vi "KeyDown.vi"(6 "PlatMods":T9, 7 "Type":T1, 8 "error in":errorcluster, 9 "VKey":T10, 10 "Char":i16, 11 "Data in":T2={"Class"={"Ants"=refnum, "Layer"=refnum, "Templates"=refnum, "Icon"=refnum, "Glyph"=refnum, "Settings"=refnum, "Tools"=refnum, "History"=refnum}, "Ref"={"Add Layer"=refnum, "Remove Layer"=refnum, "Line Text"=[], "Body Text Spec"=refnum, "DNL_Font"=refnum, "glyph path str"=refnum, "templates path str"=refnum, "Arrow Up"=refnum, "Arrow Down"=refnum, "IE VI Ref"=refnum, "Glyphs tree"=refnum, "Templates tree"=refnum, "Layer Icon Text"=refnum, "Layer Template"=refnum, "Body Text"=refnum, "Search Templates"=refnum, "TextMarker"=refnum, "Tab Control"=refnum, "Search Glyphs"=refnum, "Line Color"=refnum, "DNL_Glyphs []"=refnum, "Fill Color"=refnum, "Tools"=refnum, "Icon"=refnum, "Preview"=refnum, "Ants"=refnum, "Terminals"=refnum, "menu reference"=refnum, "LayerNames"=[], "GlyphLoadAnimation"=refnum, "TemplateLoadAnimation"=refnum, "refreshGlyphs"=refnum, "refreshTemplates"=refnum}, "Support"={"AntsRect"={"left"=0, "top"=0, "right"=0, "bottom"=0}, "Mouse Move Coords"={"Horizontal"=0, "Vertical"=0}, "Mouse Down Coords"={"Horizontal"=0, "Vertical"=0}, "Temp Coord"={"Horizontal"=0, "Vertical"=0}, "Action"=enum."Default", "Edge Color"=4914962, "Fill Color"=16860, "Mouse Down?"=FALSE, "Draft Mode?"=FALSE, "Temp Icon"=bytes[3102], "CTRL Pressed"=FALSE, "Move Selection?"=FALSE, "AntsRect Orig"={"left"=0, "top"=0, "right"=0, "bottom"=0}, "Text"="", "TM Set?"=FALSE, "Mouse inside icon?"=FALSE, "Tool (old value)"=0, "Pencil Move Color"=0, "Swap Colors?"=FALSE, "Shift pressed?"=FALSE}}) -> (0 "error out":errorcluster, 1 "Discard?":bool, 3 "Data out":T2={"Class"={"Ants"=refnum, "Layer"=refnum, "Templates"=refnum, "Icon"=refnum, "Glyph"=refnum, "Settings"=refnum, "Tools"=refnum, "History"=refnum}, "Ref"={"Add Layer"=refnum, "Remove Layer"=refnum, "Line Text"=[], "Body Text Spec"=refnum, "DNL_Font"=refnum, "glyph path str"=refnum, "templates path str"=refnum, "Arrow Up"=refnum, "Arrow Down"=refnum, "IE VI Ref"=refnum, "Glyphs tree"=refnum, "Templates tree"=refnum, "Layer Icon Text"=refnum, "Layer Template"=refnum, "Body Text"=refnum, "Search Templates"=refnum, "TextMarker"=refnum, "Tab Control"=refnum, "Search Glyphs"=refnum, "Line Color"=refnum, "DNL_Glyphs []"=refnum, "Fill Color"=refnum, "Tools"=refnum, "Icon"=refnum, "Preview"=refnum, "Ants"=refnum, "Terminals"=refnum, "menu reference"=refnum, "LayerNames"=[], "GlyphLoadAnimation"=refnum, "TemplateLoadAnimation"=refnum, "refreshGlyphs"=refnum, "refreshTemplates"=refnum}, "Support"={"AntsRect"={"left"=0, "top"=0, "right"=0, "bottom"=0}, "Mouse Move Coords"={"Horizontal"=0, "Vertical"=0}, "Mouse Down Coords"={"Horizontal"=0, "Vertical"=0}, "Temp Coord"={"Horizontal"=0, "Vertical"=0}, "Action"=enum."Default", "Edge Color"=4914962, "Fill Color"=16860, "Mouse Down?"=FALSE, "Draft Mode?"=FALSE, "Temp Icon"=bytes[3102], "CTRL Pressed"=FALSE, "Move Selection?"=FALSE, "AntsRect Orig"={"left"=0, "top"=0, "right"=0, "bottom"=0}, "Text"="", "TM Set?"=FALSE, "Mouse inside icon?"=FALSE, "Tool (old value)"=0, "Pencil Move Color"=0, "Swap Colors?"=FALSE, "Shift pressed?"=FALSE}})   [LabVIEW 2020]
uses:
  Class/Ants/Ants.lvclass
  Class/FakedArray/FakedArray.lvclass
  vi.lib/LabVIEW Icon API/lv_icon/Classes/Icon/Icon.lvclass
  Class/Icon Library/Glyph.lvclass
  Class/Settings/Settings.lvclass
  Class/Tools/Tools Paint.lvclass
  History/History/History.lvclass
  lv_icon.lvlib
  <vilib>/Utility/miscctls.llb/LVPoint32TypeDef.ctl
  <vilib>/event_ctls.llb/lveventtype.ctl
  Controls/SupportClass_Action.ctl
  History/History.lvlib
  <vilib>/event_ctls.llb/eventvkey.ctl
  Controls/Support Cluster.ctl
  Controls/References Cluster.ctl
  Controls/IE Classes.ctl
  Controls/Global Data.ctl
  vi.lib/LabVIEW Icon API/lv_icon/Controls/IEColor.ctl
panel:
  in  "Layer name":string="Clipboard"
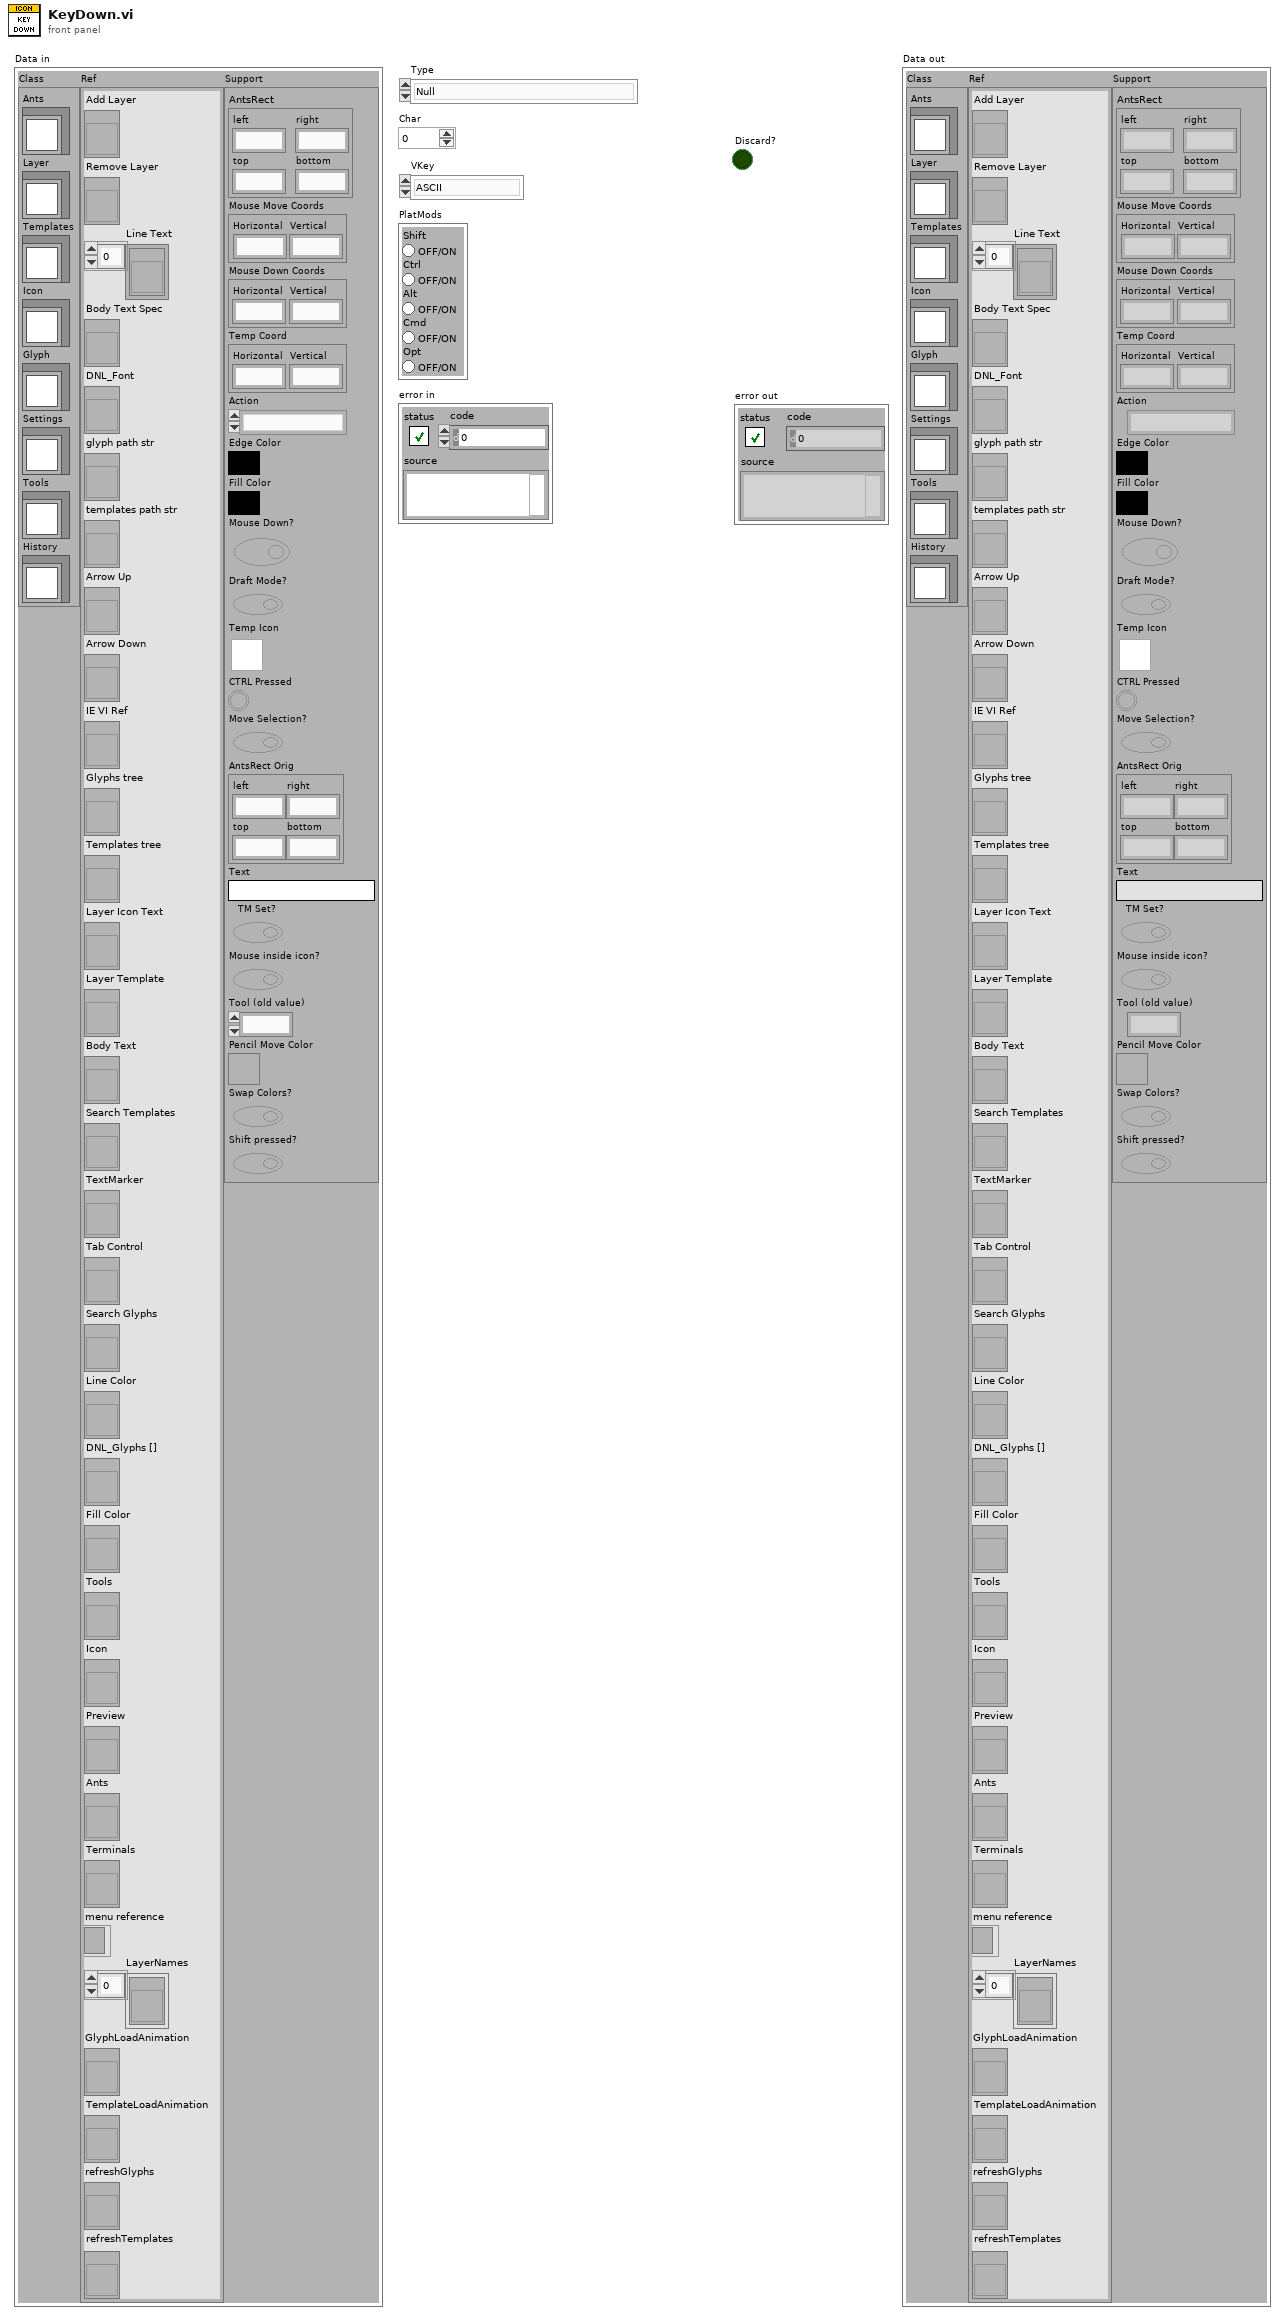
[diagram p1: front panel]
types:
  T1 = typedef "lveventtype.ctl" = enum32{"Null", "Timeout", "Annotation Menu Selection", "Annotation Menu Selection?", "App Instance Close", "App Instance Close?", "Autoscale Range Change", "Bookmark Info Change", "Cell Edit", "Cell Edit?", "Cursor Grab", "Cursor Grab?", "Cursor Menu Selection", "Cursor Menu Selection?", "Cursor Move", "Cursor Release", "Data Change", "Direction Change", "Display State Change", "Drag Ended", "Drag Enter", "Drag Leave", "Drag Over", "Drag Source Update", "Drag Starting", "Drag Starting?", "Drop", "Exec State Change", "Key Down", "Key Down?", "Key Repeat", "Key Repeat?", "Key Up", "Listbox Double Click", "Menu Activation?", "Menu Selection (App)", "Menu Selection? (App)", "Menu Selection (User)", "Mouse Down", "Mouse Down?", "Mouse Enter", "Mouse Leave", "Mouse Move", "Mouse Up", "Mouse Wheel", "NI Security User Change (App)", "Pane Size", "Panel Close", "Panel Close?", "Panel Resize", "Plot Attribute Change", "Scale Range Change", "Shortcut Menu Activation?", "Shortcut Menu Selection (App)", "Shortcut Menu Selection? (App)", "Shortcut Menu Selection (User)", "Tree Double Click", "Tree Drag", "Tree Drag?", "Tree Drop", "Tree Drop?", "Tree Item Close", "Tree Item Close?", "Tree Item Open", "Tree Item Open?", "URL Change?", "User Event", "Value Change"}
  T2 = typedef "lv_icon.lvlib/Global Data.ctl" = cluster{"Class":T3, "Ref":T4, "Support":T5}
  T3 = typedef "lv_icon.lvlib/IE Classes.ctl" = cluster{"Ants":refnum<class "Ants.lvclass">, "Layer":refnum<class "FakedArray.lvclass">, "Templates":refnum<class "FakedArray.lvclass">, "Icon":refnum<class "Icon.lvclass">, "Glyph":refnum<class "Glyph.lvclass">, "Settings":refnum<class "Settings.lvclass">, "Tools":refnum<class "Tools Paint.lvclass">, "History":refnum<class "History.lvclass">}
  T4 = typedef "lv_icon.lvlib/References Cluster.ctl" = cluster{"Add Layer":refnum<vi>, "Remove Layer":refnum<vi>, "Line Text":refnum<vi>[], "Body Text Spec":refnum<vi>, "DNL_Font":refnum<vi>, "glyph path str":refnum<vi>, "templates path str":refnum<vi>, "Arrow Up":refnum<vi>, "Arrow Down":refnum<vi>, "IE VI Ref":refnum<vi>, "Glyphs tree":refnum<vi>, "Templates tree":refnum<vi>, "Layer Icon Text":refnum<vi>, "Layer Template":refnum<vi>, "Body Text":refnum<vi>, "Search Templates":refnum<vi>, "TextMarker":refnum<vi>, "Tab Control":refnum<vi>, "Search Glyphs":refnum<vi>, "Line Color":refnum<vi>, "DNL_Glyphs []":refnum<vi>, "Fill Color":refnum<vi>, "Tools":refnum<vi>, "Icon":refnum<vi>, "Preview":refnum<vi>, "Ants":refnum<vi>, "Terminals":refnum<vi>, "menu reference":refnum<k9>, "LayerNames":refnum<vi>[], "GlyphLoadAnimation":refnum<vi>, "TemplateLoadAnimation":refnum<vi>, "refreshGlyphs":refnum<vi>, "refreshTemplates":refnum<vi>}
  T5 = typedef "lv_icon.lvlib/Support Cluster.ctl" = cluster{"AntsRect":cluster{"left":i16, "top":i16, "right":i16, "bottom":i16}, "Mouse Move Coords":T6, "Mouse Down Coords":T6, "Temp Coord":T6, "Action":T7, "Edge Color":T8, "Fill Color":T8, "Mouse Down?":bool, "Draft Mode?":bool, "Temp Icon":picture, "CTRL Pressed":bool, "Move Selection?":bool, "AntsRect Orig":cluster{"left":i16, "top":i16, "right":i16, "bottom":i16}, "Text":string, "TM Set?":bool, "Mouse inside icon?":bool, "Tool (old value)":u32, "Pencil Move Color":u32, "Swap Colors?":bool, "Shift pressed?":bool}
  T6 = typedef "LVPoint32TypeDef.ctl" = cluster{"Horizontal":i32, "Vertical":i32}
  T7 = typedef "SupportClass_Action.ctl" = enum16{"Default", "Move Selection", "Glyph Library", "Tool"}
  T8 = typedef "IEColor.ctl" = u32
  T9 = cluster{"Shift":bool, "Ctrl":bool, "Alt":bool, "Cmd":bool, "Opt":bool}
  T10 = typedef "eventvkey.ctl" = enum16{"ASCII", "Enter", "Return", "Shift", "Ctrl", "Alt", "Cmd", "Opt", "Caps", "NumLock", "Clear", "Break", "Up", "Down", "Left", "Right", "Insert", "Delete", "Home", "End", "PageUp", "PageDown", "Escape", "Help", "Pause", "ScrollLock", "F1", "F2", "F3", "F4", "F5", "F6", "F7", "F8", "F9", "F10", "F11", "F12", "F13", "F14", "F15", "F16", "F17", "F18", "F19", "F20", "F21", "F22", "F23", "F24", "Play", "VolumeUp", "VolumeDown", "Mute", "Two Byte Char"}
  T11 = cluster{"left":i16, "top":i16, "right":i16, "bottom":i16}
  T12 = enum32{"Pencil", "Line", "Dropper", "Fill", "Rectangle", "Filled Rectangle", "Ellipse", "Filled Ellipse", "Eraser", "Text", "Select", "Move"}
  T13 = typedef "Graphic.ctl" = cluster{"Rectangle":cluster{"left":i16, "top":i16, "right":i16, "bottom":i16}, "Path":path, "Image":picture, "Filter":string, "FileName":string}
  T14 = cluster{"left":i16, "top":i16, "bottom":i16, "right":i16}
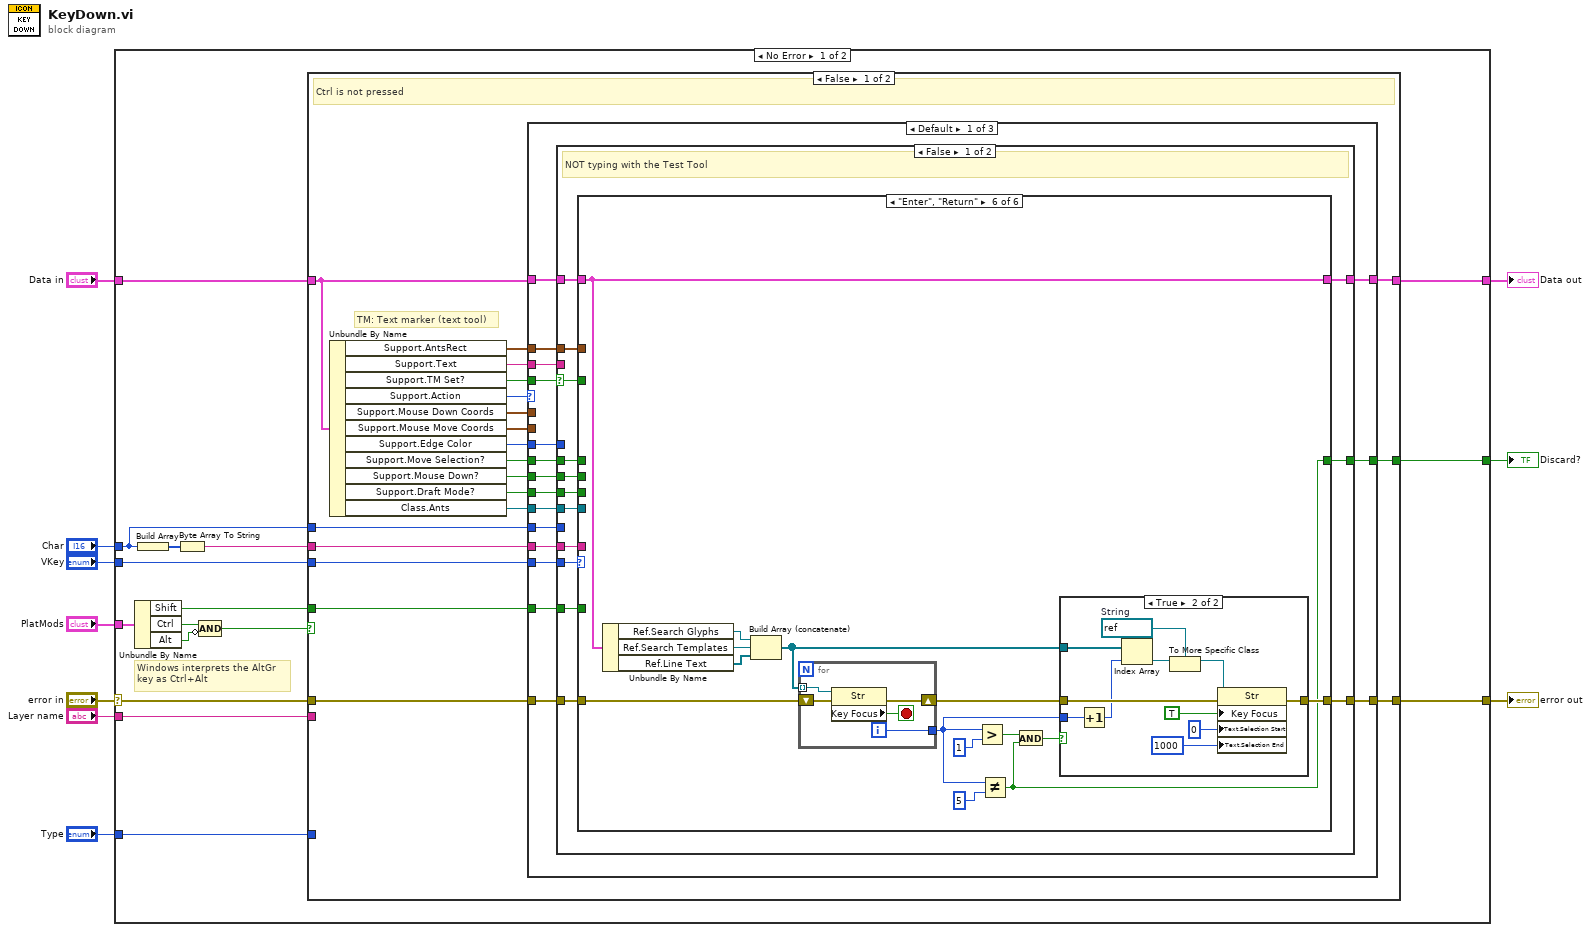
[diagram p0: block diagram]
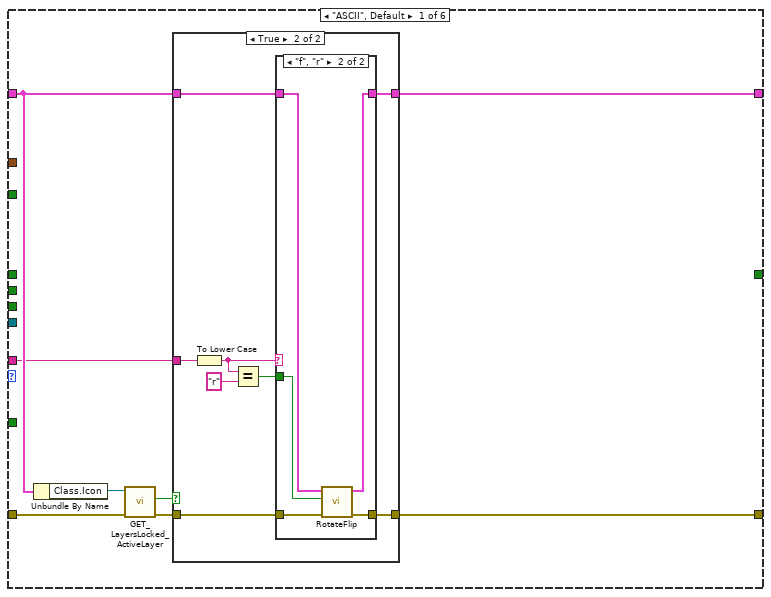
[diagram p2: hidden frame]
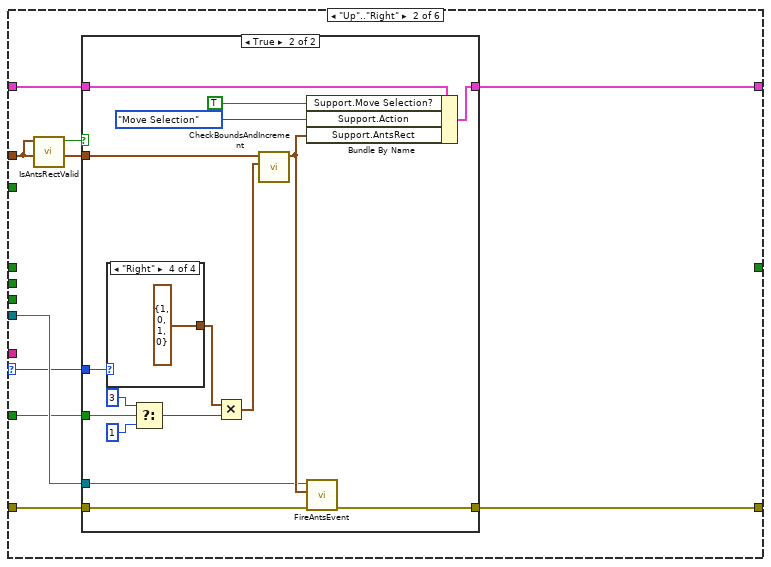
[diagram p5: hidden frame]
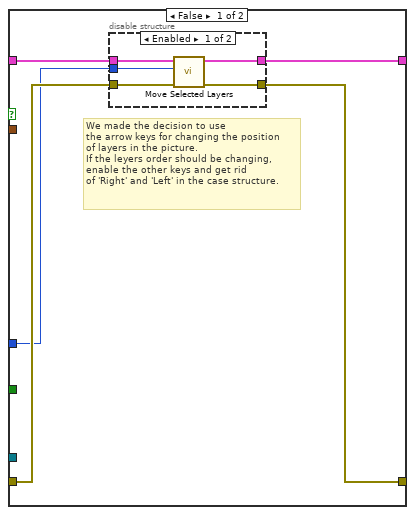
[diagram p6: hidden frame]
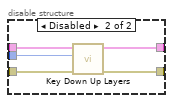
[diagram p7: hidden frame]
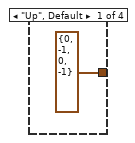
[diagram p8: hidden frame]
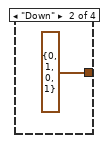
[diagram p9: hidden frame]
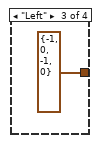
[diagram p10: hidden frame]
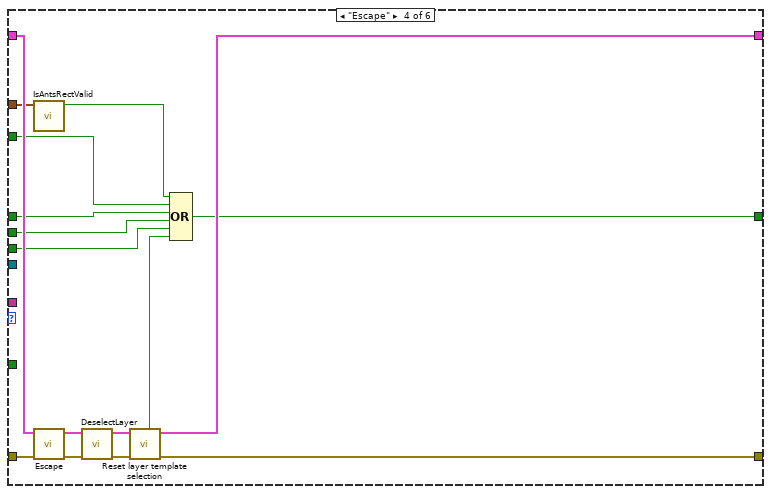
[diagram p12: hidden frame]
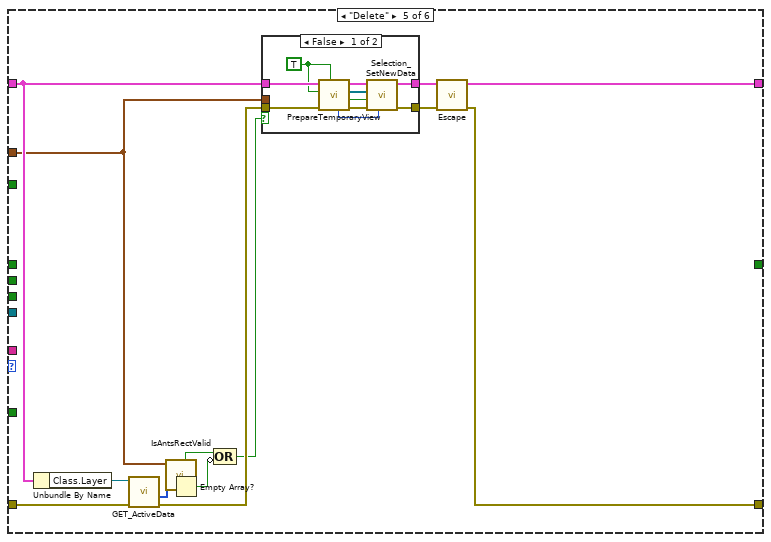
[diagram p13: hidden frame]
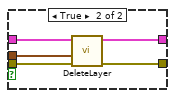
[diagram p14: hidden frame]
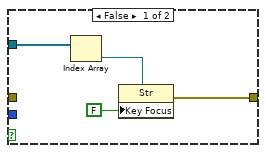
[diagram p15: hidden frame]
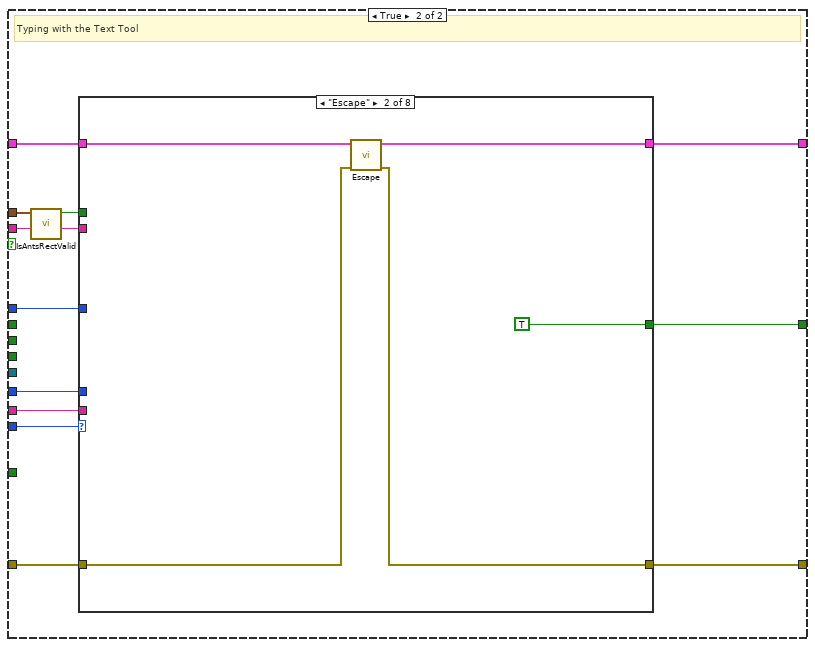
[diagram p16: hidden frame]
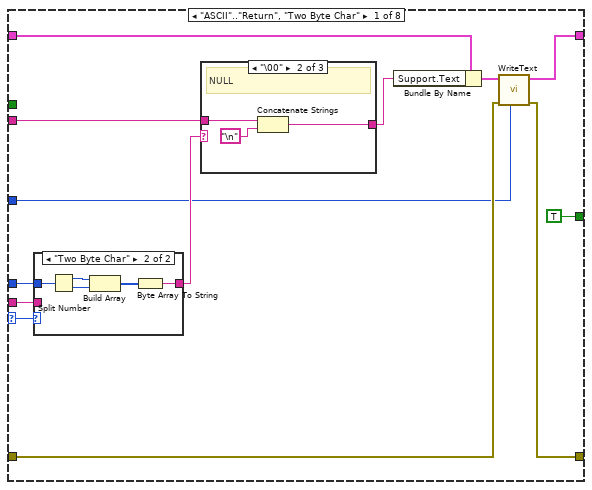
[diagram p17: hidden frame]
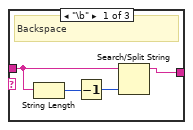
[diagram p19: hidden frame]
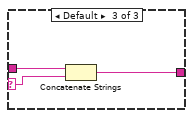
[diagram p20: hidden frame]
diagram:
  n1 = case shown="No Error" "error in" {
    selector: "error in" -> [w25 w688]
    tunnel: [w26 w688] -> w9
    tunnel: "VKey" -> [w24 _]
    tunnel: "Char" -> [w18 _]
    tunnel: "PlatMods" -> [w15 _]
    tunnel: [w21 _] -> w5
    tunnel: "Data in" -> [w16 w687]
    tunnel: [w20 w687] -> w3
    tunnel: "Type" -> [w19 _]
    tunnel: "Layer name" -> [w17 _]
    frame No Error {
      # "Windows interprets the AltGr\nkey as Ctrl+Alt"
      n2 = Unbundle By Name(w15) -> ("Shift"=w11:bool, "Ctrl"=w12:bool, "Alt"=w14:bool)
      n3 = Build Array(w18) -> (w23:i16[])
      n4 = Byte Array To String(unsigned byte array=w23) -> (string=w22:string)
      n5 = Compound Arithmetic op=AND(w12, invert w14) -> (w13:bool)
      n6 = case shown="False" w13 {
        selector: w13 -> [_ w489]
        tunnel: w24 -> [w44 _]
        tunnel: w22 -> [w43 w487]
        tunnel: [w45 w499] -> w26
        tunnel: [w32 w486] -> w21
        tunnel: w25 -> [w46 w500]
        tunnel: w16 -> [w31 w481]
        tunnel: [w29 w498] -> w20
        tunnel: w19 -> [_ w493]
        tunnel: w18 -> [w28 _]
        tunnel: w17 -> [_ w484]
        tunnel: w11 -> [w27 w482]
        frame False {
          # "TM: Text marker (text tool)"
          # "Ctrl is not pressed"
          n7 = Unbundle By Name(w31) -> ("Support.AntsRect"=w37:T11, "Support.Text"=w40:string, "Support.TM Set?"=w41:bool, "Support.Action"=w42:T7, "Support.Mouse Down Coords"=w39:T6, "Support.Mouse Move Coords"=w36:T6, "Support.Edge Color"=w38:T8, "Support.Move Selection?"=w35:bool, "Support.Mouse Down?"=w34:bool, "Support.Draft Mode?"=w33:bool, "Class.Ants"=w30:refnum<class "Ants.lvclass">)
          n8 = case shown="Default" w42 {
            tunnel: w44 -> [w61 w333 w400]
            tunnel: w43 -> [w58 w332 _]
            tunnel: w46 -> [w62 w335 w402]
            tunnel: [w63 w334 w401] -> w45
            tunnel: w41 -> [w60 w330 w398]
            tunnel: w40 -> [w59 _ _]
            tunnel: w39 -> [_ _ _]
            tunnel: w38 -> [w57 _ _]
            tunnel: w37 -> [w56 w331 w399]
            tunnel: w36 -> [_ w323 _]
            tunnel: w35 -> [w55 w329 w397]
            tunnel: w34 -> [w54 w328 w396]
            tunnel: w33 -> [w53 w327 w395]
            tunnel: [w52 w326 w394] -> w32
            tunnel: w27 -> [w51 _ w390]
            tunnel: w31 -> [w50 w325 w393]
            tunnel: [w49 w324 w392] -> w29
            tunnel: w30 -> [w47 _ w391]
            tunnel: w28 -> [w48 _ _]
            frame Default {
              n9 = case shown="False" w60 {
                selector: w60 -> [w69 _]
                tunnel: w61 -> [w75 w236]
                tunnel: [w76 w238] -> w63
                tunnel: w62 -> [w77 w237]
                tunnel: w59 -> [_ w235]
                tunnel: w58 -> [w74 w234]
                tunnel: w57 -> [_ w231]
                tunnel: w56 -> [w73 w233]
                tunnel: w55 -> [w72 _]
                tunnel: w54 -> [w71 _]
                tunnel: w53 -> [w70 _]
                tunnel: [w68 w230] -> w52
                tunnel: w51 -> [w67 _]
                tunnel: w50 -> [w66 w229]
                tunnel: [w65 w228] -> w49
                tunnel: w48 -> [_ w227]
                tunnel: w47 -> [w64 _]
                frame False {
                  # "NOT typing with the Test Tool"
                  n10 = case shown="\"Enter\", \"Return\"" w75 {
                    selector: w75 -> [_ w108 _ _ _ _]
                    tunnel: w77 -> [w84 w111 w148 w164 w175 w206]
                    tunnel: [w85 w110 w148 w161 w177 w204] -> w76
                    tunnel: w74 -> [w78 _ _ _ _ _]
                    tunnel: w73 -> [_ w103 _ w158 w165 _]
                    tunnel: w72 -> [_ _ _ w156 _ _]
                    tunnel: w71 -> [_ _ _ w155 _ _]
                    tunnel: w70 -> [_ _ _ w154 _ _]
                    tunnel: w69 -> [_ _ _ w157 _ _]
                    tunnel: [_ _ _ w149 _ w194] -> w68
                    tunnel: w67 -> [_ w107 _ _ _ _]
                    tunnel: w66 -> [w82 w106 w147 w160 w171 w203]
                    tunnel: [w81 w105 w147 w151 w173 w203] -> w65
                    tunnel: w64 -> [_ w109 _ _ _ _]
                    frame "ASCII", Default {
                      n11 = Unbundle By Name(w82) -> ("Class.Icon"=w80:refnum<class "Icon.lvclass">)
                      n12 = call-dynamic "GET_LayersLocked_ActiveLayer.vi"("error in (no error)"=w84, "Icon.lvclass in"=w80) -> ("error out"=w83:errorcluster, "Layers Locked?"=w79:bool)  [unwired: 8 out]
                      n13 = case shown="True" w79 {
                        tunnel: w78 -> [_ w92]
                        tunnel: w83 -> [w87 w95]
                        tunnel: [w87 w94] -> w85
                        tunnel: w82 -> [w86 w89]
                        tunnel: [w86 w88] -> w81
                        frame False {
                        }
                        frame True {
                          n14 = To Lower Case(string=w92) -> (all lower case string=w90:string)
                          n15 = Equal?(x=w90, y="r") -> (x = y?=w91:bool)
                          n16 = case shown="\"f\", \"r\"" w90 {
                            tunnel: w95 -> [w97 w102]
                            tunnel: [w97 w101] -> w94
                            tunnel: w91 -> [_ w100]
                            tunnel: w89 -> [w96 w99]
                            tunnel: [w96 w98] -> w88
                            frame Default {
                            }
                            frame "f", "r" {
                              n17 = call "RotateFlip.vi"("error in"=w102, "Rotate"=w100, "Data in"=w99) -> ("error out"=w101:errorcluster, "Data out"=w98:T2)  [unwired: 3 in, 4 out]
                            }
                          }
                        }
                      }
                    }
                    frame "Up".."Right" {
                      n18 = call "IsAntsRectValid.vi"("AntsRect"=w103) -> ("Valid?"=w104:bool)  [unwired: 10 out]
                      n19 = case shown="True" w104 {
                        tunnel: w111 -> [w116 w141]
                        tunnel: [w115 w142] -> w110
                        tunnel: w108 -> [w114 w130]
                        tunnel: w107 -> [_ w129]
                        tunnel: w106 -> [w113 w138]
                        tunnel: [w112 w136] -> w105
                        tunnel: w103 -> [_ w127]
                        tunnel: w109 -> [_ w128]
                        frame False {
                          # "We made the decision to use\nthe arrow keys for changing the position\nof layers in the picture.\nIf the leyers order should be changing,\nenable the other keys and get rid\nof 'Right' and 'Left' in the case structure."
                          n20 = disable-structure shown="Enabled" {
                            disable-tunnel: w116 -> [w121 w126]
                            disable-tunnel: [w120 w125] -> w115
                            disable-tunnel: w114 -> [w117 w122]
                            disable-tunnel: w113 -> [w119 w124]
                            disable-tunnel: [w118 w123] -> w112
                            frame Enabled {
                              n21 = call "Move Selected Layers.vi"("error in"=w121, "VKey"=w117, "Data in"=w119) -> ("error out"=w120:errorcluster, "Data out"=w118:T2)  [unwired: 1 in, 6 out]
                            }
                            frame Disabled {
                              n22 = call "Key Down Up Layers.vi"("error in"=w126, "VKey"=w122, "Data in"=w124) -> ("error out"=w125:errorcluster, "Data out"=w123:T2)  [unwired: 1 in, 6 out]
                            }
                          }
                        }
                        frame True {
                          n23 = case shown="\"Right\"" w130 {
                            tunnel: [T11 {"left"=0, "top"=-1, "right"=0, "bottom"=-1} ("y") T11 {"left"=0, "top"=1, "right"=0, "bottom"=1} ("y") T11 {"left"=-1, "top"=0, "right"=-1, "bottom"=0} ("y") T11 {"left"=1, "top"=0, "right"=1, "bottom"=0} ("y")] -> w134
                            frame "Up", Default {
                            }
                            frame "Down" {
                            }
                            frame "Left" {
                            }
                            frame "Right" {
                            }
                          }
                          n24 = Select(t=i16 3 ("left"), s=w129, f=i16 1 ("left")) -> (s? t:f=w131:i16)
                          n25 = Multiply(x=w134, y=w131) -> (x*y=w139:T11)
                          n26 = call "CheckBoundsAndIncrement.vi"("Increment"=w139, "Rectangle In"=w127) -> ("Rectangle Out"=w140:T11)  [unwired: 9 in]
                          n27 = Bundle By Name(cluster=w138, "Support.Move Selection?"=TRUE, "Support.Action"=SupportClass_Action."Move Selection", "Support.AntsRect"=w140) -> (w136:T2)
                          n28 = call "FireAntsEvent.vi"("error in (no error)"=w141, "Rectangle (default: deselect)"=w140, "Ants in"=w128) -> ("error out"=w142:errorcluster)  [unwired: 1 in, 7 out]
                        }
                      }
                    }
                    frame "Shift" {
                    }
                    frame "Escape" {
                      n29 = call "IsAntsRectValid.vi"("AntsRect"=w158) -> ("Valid?"=w159:bool)  [unwired: 10 out]
                      n30 = call "Escape.vi"("error in"=w164, "Data in"=w160) -> ("error out"=w163:errorcluster, "Data out"=w153:T2)  [unwired: 8 out]
                      n31 = call "DeselectLayer.vi"("error in (no error)"=w163, "Data in"=w153) -> ("error out"=w162:errorcluster, "Data out"=w152:T2)  [unwired: 8 out]
                      n32 = call "Reset layer template selection.vi"("error in (no error)"=w162, "Data in"=w152) -> ("error out"=w161:errorcluster, "Data out"=w151:T2, "Layers selected?"=w150:bool)  [unwired: 1 in, 6 out]
                      n33 = Compound Arithmetic op=OR(w159, w157, w156, w155, w154, w150) -> (w149:bool)
                    }
                    frame "Delete" {
                      n34 = Unbundle By Name(w171) -> ("Class.Layer"=w172:refnum<class "FakedArray.lvclass">)
                      n35 = call-dynamic "GET_ActiveData.vi"("error in (no error)"=w175, "FakedArray in"=w172) -> ("error out"=w174:errorcluster, "Active Data []"=w170:i32[])  [unwired: 4 in, 4 out]
                      n36 = call "IsAntsRectValid.vi"("AntsRect"=w165) -> ("Max. Rect size?"=w166:bool)  [unwired: 10 out]
                      n37 = Empty Array?(array=w170) -> (empty?=w169:bool)
                      n38 = Compound Arithmetic op=OR(w166, invert w169) -> (w168:bool)
                      n39 = case shown="False" w168 {
                        tunnel: w171 -> [w184 w190]
                        tunnel: [w187 w192] -> w176
                        tunnel: [w183 w189] -> w167
                        tunnel: w174 -> [w185 w191]
                        tunnel: w165 -> [_ w188]
                        frame False {
                          w182 = TRUE ("Delete Selected Area?")
                          n40 = call "PrepareTemporaryView.vi"("Delete Selected Area?"=w182, "error in (no error)"=w185, "Valid Selection?"=w182, "Data in"=w184) -> ("error out"=w186:errorcluster, "Highlighted?"=w180:bool, "All Layers out"=w181:refnum<class "Layer.lvclass">[], "Data out"=w178:T2, "#Active Layer"=w179:i32)  [unwired: 1 in, 2 out]
                          n41 = call "Selection_SetNewData.vi"("#Active Layer"=w179, "error in"=w186, "Highlighted?"=w180, "All Layers In"=w181, "Data in"=w178) -> ("error out"=w187:errorcluster, "Data out"=w183:T2)  [unwired: 1 in, 3 out]
                        }
                        frame True {
                          n42 = call "DeleteLayer.vi"("error in"=w191, "AntsRect"=w188, "Data in"=w190) -> ("error out"=w192:errorcluster, "Data out"=w189:T2)  [unwired: 5 out]
                        }
                      }
                      n43 = call "Escape.vi"("error in"=w176, "Data in"=w167) -> ("error out"=w177:errorcluster, "Data out"=w173:T2)  [unwired: 8 out]
                    }
                    frame "Enter", "Return" {
                      n44 = Unbundle By Name(w203) -> ("Ref.Search Glyphs"=w198:refnum<vi>, "Ref.Search Templates"=w199:refnum<vi>, "Ref.Line Text"=w201:refnum<vi>[])
                      n45 = Build Array (concatenate)(w198, w199, w201) -> (w200:refnum<vi>[])
                      n46 = for {
                        tunnel: w200 -> [w224] mode=indexing
                        shift-right: [w226] -> w205
                        shift-left: w206 -> [w225]
                        tunnel: [w223] -> w197
                        i -> [w223]
                        stop <- w222 stop-if-true
                        n47 = property class="Str"(reference=w224, error in=w225) -> (error out=w226:errorcluster, "Key Focus"=w222:bool)  [unwired: 1 out]
                      }
                      n48 = Greater?(x=w197, y=1) -> (0:w195:bool)
                      n49 = Not Equal?(x=w197, y=5) -> (x != y?=w194:bool)
                      n50 = And(x=w195, y=w194) -> (x .and. y?=w193:bool)
                      n51 = case shown="True" w193 {
                        tunnel: w197 -> [_ w218]
                        tunnel: w200 -> [w209 w219]
                        tunnel: w205 -> [_ w221]
                        tunnel: [w210 w220] -> w204
                        frame False {
                          n52 = Index Array(array=w209) -> (element=w208:refnum<vi>)  [unwired: 1 in]
                          n53 = property class="Str"(reference=w208, "Key Focus"=FALSE) -> (error out=w210:errorcluster)  [unwired: 1 in, 1 out]
                        }
                        frame True {
                          w211 = refnum<vi> refnum  # String
                          n54 = Increment(x=w218) -> (x+1=w217:i32)
                          n55 = Index Array(array=w219, index=w217) -> (element=w216:refnum<vi>)
                          n56 = To More Specific Class(target class=w211, reference=w216) -> (specific class reference=w212:refnum<vi>)  [unwired: 1 in, 1 out]
                          n57 = property class="Str"(reference=w212, error in=w221, "Key Focus"=TRUE, "Text.Selection Start"=u32 0 ("Text.Selection:Start"), "Text.Selection End"=u32 1000 ("Text.Selection:End")) -> (error out=w220:errorcluster)  [unwired: 1 out]
                        }
                      }
                    }
                  }
                }
                frame True {
                  # "Typing with the Text Tool"
                  n58 = call "IsAntsRectValid.vi"("AntsRect"=w233) -> ("Valid?"=w232:bool)  [unwired: 10 out]
                  n59 = case shown="\"Escape\"" w236 {
                    selector: w236 -> [w243 _ _ _ _ _ _ _]
                    tunnel: [w250 w272 w274 w279 w303 w309 w315 w321] -> w238
                    tunnel: w237 -> [w251 w271 w274 w280 w304 w310 w316 w322]
                    tunnel: w235 -> [w249 _ _ w278 _ _ _ _]
                    tunnel: w234 -> [w241 _ _ _ _ _ _ _]
                    tunnel: w231 -> [w239 _ _ _ w302 w308 w314 w320]
                    tunnel: w232 -> [_ _ _ w277 _ _ _ _]
                    tunnel: [TRUE TRUE _ _ _ _ _ _] -> w230
                    tunnel: w229 -> [w244 w269 w273 w276 w301 w306 w313 w319]
                    tunnel: [w247 w268 w273 w275 w299 w305 w312 w317] -> w228
                    tunnel: w227 -> [w240 _ _ _ _ _ _ _]
                    frame "ASCII".."Return", "Two Byte Char" {
                      n60 = case shown="\"Two Byte Char\"" w243 {
                        tunnel: [w252 w253] -> w242
                        tunnel: w241 -> [w252 _]
                        tunnel: w240 -> [_ w257]
                        frame "ASCII", Default {
                        }
                        frame "Two Byte Char" {
                          n61 = Split Number(x=w257) -> (hi(x)=w255:u8, lo(x)=w256:u8)
                          n62 = Build Array(w255, w256) -> (w254:u8[])
                          n63 = Byte Array To String(unsigned byte array=w254) -> (string=w253:string)
                        }
                      }
                      n64 = case shown="\"\\00\"" w242 {
                        selector: w242 -> [_ _ w265]
                        tunnel: w249 -> [w259 w264 w267]
                        tunnel: [w258 w263 w266] -> w246
                        frame "\b" {
                          # "Backspace"
                          n65 = String Length(string=w259) -> (length=w261:i32)
                          n66 = Decrement(x=w261) -> (x-1=w260:i32)
                          n67 = Search/Split String(string=w259, offset (0)=w260) -> (substring before match=w258:string)  [unwired: 3 out]
                        }
                        frame "\u0000\u0000" {
                          # "NULL"
                          n68 = Concatenate Strings(w264, "\n") -> (w263:string)
                        }
                        frame Default {
                          n69 = Concatenate Strings(w267, w265) -> (w266:string)
                        }
                      }
                      n70 = Bundle By Name(cluster=w244, "Support.Text"=w246) -> (w245:T2)
                      n71 = call "WriteText.vi"("Text Color"=w239, "error in (no error)"=w251, "Data in"=w245) -> ("error out"=w250:errorcluster, "Data out"=w247:T2)  [unwired: 2 in, 5 out]
                    }
                    frame "Escape" {
                      n72 = call "Escape.vi"("error in"=w271, "Data in"=w269) -> ("error out"=w272:errorcluster, "Data out"=w268:T2)  [unwired: 8 out]
                    }
                    frame Default {
                    }
                    frame "Delete" {
                      n73 = case shown="True" w277 {
                        tunnel: w278 -> [_ _]
                        tunnel: w280 -> [w282 w295]
                        tunnel: [w282 w297] -> w279
                        tunnel: w276 -> [w281 w285]
                        tunnel: [w281 w286] -> w275
                        frame False {
                        }
                        frame True {
                          w292 = TRUE ("Delete Selected Area?")
                          n74 = call "PrepareTemporaryView.vi"("Delete Selected Area?"=w292, "error in (no error)"=w295, "Valid Selection?"=w292, "Data in"=w285) -> ("error out"=w298:errorcluster, "Highlighted?"=w290:bool, "All Layers out"=w291:refnum<class "Layer.lvclass">[], "Data out"=w288:T2, "#Active Layer"=w289:i32)  [unwired: 1 in, 2 out]
                          n75 = call "Selection_SetNewData.vi"("#Active Layer"=w289, "error in"=w298, "Highlighted?"=w290, "All Layers In"=w291, "Data in"=w288) -> ("error out"=w296:errorcluster, "Data out"=w287:T2)  [unwired: 1 in, 3 out]
                          n76 = call "ViewLayer.vi"("error in (no error)"=w296, "Data in"=w287) -> ("error out"=w294:errorcluster, "Data out"=w284:T2)  [unwired: 3 in, 5 out]
                          n77 = call "Set Undo Flag.vi"("error in"=w294, "Data in"=w284) -> ("error out"=w293:errorcluster, "Data out"=w283:T2)  [unwired: 8 in]
                          n78 = call "Escape.vi"("error in"=w293, "Data in"=w283) -> ("error out"=w297:errorcluster, "Data out"=w286:T2)  [unwired: 8 out]
                        }
                      }
                    }
                    frame "Up" {
                      n79 = call "WriteText.vi"("Text Color"=w302, "error in (no error)"=w304, "Offset"=T6 {"Horizontal"=0, "Vertical"=-1} ("y"), "Data in"=w301) -> ("error out"=w303:errorcluster, "Data out"=w299:T2)  [unwired: 1 in, 5 out]
                    }
                    frame "Down" {
                      n80 = call "WriteText.vi"("Text Color"=w308, "error in (no error)"=w310, "Offset"=T6 {"Horizontal"=0, "Vertical"=1} ("y"), "Data in"=w306) -> ("error out"=w309:errorcluster, "Data out"=w305:T2)  [unwired: 1 in, 5 out]
                    }
                    frame "Left" {
                      n81 = call "WriteText.vi"("Text Color"=w314, "error in (no error)"=w316, "Offset"=T6 {"Horizontal"=-1, "Vertical"=0} ("y"), "Data in"=w313) -> ("error out"=w315:errorcluster, "Data out"=w312:T2)  [unwired: 6 out]
                    }
                    frame "Right" {
                      n82 = call "WriteText.vi"("Text Color"=w320, "error in (no error)"=w322, "Offset"=T6 {"Horizontal"=1, "Vertical"=0} ("y"), "Data in"=w319) -> ("error out"=w321:errorcluster, "Data out"=w317:T2)  [unwired: 6 out]
                    }
                  }
                }
              }
            }
            frame "Glyph Library" {
              n83 = case shown="\"ASCII\", Default" w333 {
                tunnel: w335 -> [w341 w385 w389]
                tunnel: [w340 w384 w389] -> w334
                tunnel: w332 -> [w339 _ _]
                tunnel: w331 -> [_ w381 _]
                tunnel: w330 -> [_ w380 _]
                tunnel: w329 -> [_ w379 _]
                tunnel: w328 -> [_ w378 _]
                tunnel: w327 -> [_ w377 _]
                tunnel: [_ w376 _] -> w326
                tunnel: w325 -> [w338 w375 w387]
                tunnel: [w337 w373 w386] -> w324
                tunnel: w323 -> [w336 _ _]
                frame "ASCII", Default {
                  n84 = case shown="\"F\", \"R\", \"f\", \"r\"" w339 {
                    selector: w339 -> [_ w356]
                    tunnel: w341 -> [w343 w364]
                    tunnel: [w343 w363] -> w340
                    tunnel: w338 -> [w342 w349]
                    tunnel: [w342 w346] -> w337
                    tunnel: w336 -> [_ w345]
                    frame Default {
                    }
                    frame "F", "R", "f", "r" {
                      n85 = Unbundle By Name(w349) -> ("Class.Glyph"=w350:refnum<class "Glyph.lvclass">)
                      n86 = To Lower Case(string=w356) -> (all lower case string=w344:string)
                      n87 = Equal?(x=w344, y="r") -> (x = y?=w351:bool)
                      n88 = call-dynamic "GET_ActiveGlyph.vi"("error in (no error)"=w364, "Glyph.lvclass in"=w350) -> ("error out"=w365:errorcluster, "Path & Icon"=w360:T13, "Glyph.lvclass out"=w359:refnum<class "Glyph.lvclass">)  [unwired: 7 out]
                      n89 = Unbundle By Name(w360) -> ("Image"=w362:picture, "Rectangle"=w361:T11)
                      n90 = call "Rotate Flip Image.vi"("Rotate?"=w351, "rect"=w361, "Temp Icon In"=w362) -> ("rect out"=w354:T14, "Temp Icon Out"=w355:picture)  [unwired: 7 out]
                      n91 = case shown="False" w351 {
                        tunnel: w355 -> [w370 w372]
                        tunnel: w354 -> [w369 w371]
                        tunnel: [w368 w372] -> w353
                        tunnel: [w367 w371] -> w352
                        frame False {
                          n92 = call "Rotate Flip Image.vi"("Rotate?"=TRUE, "rect"=w369, "Temp Icon In"=w370) -> ("rect out"=w367:T14, "Temp Icon Out"=w368:picture)  [unwired: 7 out]
                        }
                        frame True {
                        }
                      }
                      n93 = Bundle By Name(cluster=w360, "Image"=w353, "Rectangle"=w352) -> (w358:T13)
                      n94 = call-dynamic "SET_ActiveGlyph.vi"("error in (no error)"=w365, "Active Glyph"=w358, "Glyph in"=w359) -> ("error out"=w363:errorcluster, "Glyph out"=w348:refnum<class "Glyph.lvclass">)  [unwired: 7 out]
                      n95 = call "TemporaryGlyphView.vi"("Mouse Coords Pic"=w345, "Path & Icon"=w358) -> ("icon out"=w347:picture)  [unwired: 9 out]
                      n96 = Bundle By Name(cluster=w349, "Class.Glyph"=w348, "Support.Temp Icon"=w347) -> (w346:T2)
                    }
                  }
                }
                frame "Escape" {
                  n97 = call "IsAntsRectValid.vi"("AntsRect"=w381) -> ("Valid?"=w382:bool)  [unwired: 10 out]
                  n98 = Compound Arithmetic op=OR(w382, w380, w379, w378, w377) -> (w376:bool)
                  n99 = call "Escape.vi"("error in"=w385, "Data in"=w375) -> ("error out"=w383:errorcluster, "Data out"=w374:T2)  [unwired: 8 out]
                  n100 = call "Reset layer template selection.vi"("error in (no error)"=w383, "Data in"=w374) -> ("error out"=w384:errorcluster, "Data out"=w373:T2)  [unwired: 1 in, 7 out]
                }
                frame "Ctrl" {
                  n101 = Bundle By Name(cluster=w387, "Support.CTRL Pressed"=TRUE ("CTRL Pressed")) -> (w386:T2)
                }
              }
            }
            frame "Move Selection" {
              n102 = case shown="\"Delete\"" w400 {
                selector: w400 -> [_ w406 _ _]
                tunnel: w402 -> [w404 w413 w448 w454]
                tunnel: [w404 w412 w445 w456] -> w401
                tunnel: w399 -> [_ w408 w442 w449]
                tunnel: w398 -> [_ _ w440 _]
                tunnel: w397 -> [_ _ w439 _]
                tunnel: w396 -> [_ _ w438 _]
                tunnel: w395 -> [_ _ w437 _]
                tunnel: [_ _ w436 _] -> w394
                tunnel: w393 -> [w403 w410 w444 w450]
                tunnel: [w403 w407 w443 w453] -> w392
                tunnel: w391 -> [_ w411 w435 _]
                tunnel: w390 -> [_ w405 _ _]
                frame "ASCII", Default {
                }
                frame "Up".."Right" {
                  n103 = call "IsAntsRectValid.vi"("AntsRect"=w408) -> ("Valid?"=w409:bool)  [unwired: 10 out]
                  n104 = case shown="True" w409 {
                    tunnel: w410 -> [w414 w427]
                    tunnel: w408 -> [_ w418]
                    tunnel: [w414 w426] -> w407
                    tunnel: w406 -> [_ w420]
                    tunnel: w405 -> [_ w424]
                    tunnel: w413 -> [w415 w428]
                    tunnel: [w415 w429] -> w412
                    tunnel: w411 -> [_ w416]
                    frame False {
                    }
                    frame True {
                      n105 = case shown="\"Up\", Default" w420 {
                        tunnel: [T11 {"left"=0, "top"=-1, "right"=0, "bottom"=-1} ("y") T11 {"left"=0, "top"=1, "right"=0, "bottom"=1} ("y") T11 {"left"=-1, "top"=0, "right"=-1, "bottom"=0} ("y") T11 {"left"=1, "top"=0, "right"=1, "bottom"=0} ("y")] -> w425
                        frame "Up", Default {
                        }
                        frame "Down" {
                        }
                        frame "Left" {
                        }
                        frame "Right" {
                        }
                      }
                      n106 = Select(t=i16 3 ("left"), s=w424, f=i16 1 ("left")) -> (s? t:f=w421:i16)
                      n107 = Multiply(x=w425, y=w421) -> (x*y=w419:T11)
                      n108 = call "CheckBoundsAndIncrement.vi"("Increment"=w419, "Rectangle In"=w418) -> ("Rectangle Out"=w417:T11)  [unwired: 9 in]
                      n109 = Bundle By Name(cluster=w427, "Support.AntsRect"=w417) -> (w426:T2)
                      n110 = call "FireAntsEvent.vi"("error in (no error)"=w428, "Rectangle (default: deselect)"=w417, "Ants in"=w416) -> ("error out"=w429:errorcluster)  [unwired: 1 in, 7 out]
                    }
                  }
                }
                frame "Escape" {
                  n111 = call "IsAntsRectValid.vi"("AntsRect"=w442) -> ("Valid?"=w441:bool)  [unwired: 10 out]
                  n112 = call "FireAntsEvent.vi"("error in (no error)"=w448, "Ants in"=w435) -> ("error out"=w447:errorcluster)  [unwired: 2 in, 7 out]
                  n113 = Compound Arithmetic op=OR(w441, w440, w439, w438, w437) -> (w436:bool)
                  n114 = call "Reset layer template selection.vi"("error in (no error)"=w447, "Data in"=w444) -> ("error out"=w446:errorcluster, "Data out"=w434:T2)  [unwired: 1 in, 7 out]
                  n115 = call "Escape.vi"("error in"=w446, "Data in"=w434) -> ("error out"=w445:errorcluster, "Data out"=w443:T2)  [unwired: 8 out]
                }
                frame "Delete" {
                  n116 = call "IsAntsRectValid.vi"("AntsRect"=w449) -> ("Max. Rect size?"=w451:bool)  [unwired: 10 out]
                  n117 = case shown="True" w451 {
                    tunnel: w450 -> [w463 w469]
                    tunnel: [w466 w478] -> w455
                    tunnel: [w462 w474] -> w452
                    tunnel: w454 -> [w464 w476]
                    tunnel: w449 -> [_ w468]
                    frame False {
                      w461 = TRUE ("Delete Selected Area?")
                      n118 = call "PrepareTemporaryView.vi"("Delete Selected Area?"=w461, "error in (no error)"=w464, "Valid Selection?"=w461, "Data in"=w463) -> ("error out"=w465:errorcluster, "Highlighted?"=w459:bool, "All Layers out"=w460:refnum<class "Layer.lvclass">[], "Data out"=w457:T2, "#Active Layer"=w458:i32)  [unwired: 1 in, 2 out]
                      n119 = call "Selection_SetNewData.vi"("#Active Layer"=w458, "error in"=w465, "Highlighted?"=w459, "All Layers In"=w460, "Data in"=w457) -> ("error out"=w466:errorcluster, "Data out"=w462:T2)  [unwired: 1 in, 3 out]
                    }
                    frame True {
                      n120 = Unbundle By Name(w469) -> ("Class.Icon"=w473:refnum<class "Icon.lvclass">)
                      n121 = call-dynamic "GET_All User Layers.vi"("error in (no error)"=w476, "Icon.lvclass in"=w473) -> ("error out"=w477:errorcluster, "User Layer"=w470:refnum<class "Layer.lvclass">[])  [unwired: 7 in, 1 out]
                      n122 = Array Size(array=w470) -> (size(s)=w471:i32)
                      n123 = for {
                        N: w471 -> [_]
                        tunnel: [w479] -> w472 mode=indexing
                        i -> [w479]
                      }
                      n124 = call "Set active Layer programmatically.vi"("error in"=w477, "Active Layer []"=w472, "Data in"=w469) -> ("error out"=w475:errorcluster, "Data out"=w467:T2)  [unwired: 7 in]
                      n125 = call "DeleteLayer.vi"("error in"=w475, "AntsRect"=w468, "Data in"=w467) -> ("error out"=w478:errorcluster, "Data out"=w474:T2)  [unwired: 5 out]
                    }
                  }
                  n126 = call "Escape.vi"("error in"=w455, "Data in"=w452) -> ("error out"=w456:errorcluster, "Data out"=w453:T2)  [unwired: 8 out]
                }
              }
            }
          }
        }
        frame True {
          # "Ctrl is pressed"
          n127 = Unbundle By Name(w481) -> ("Support.AntsRect"=w483:T11, "Support.Action"=w488:T7, "Support.Mouse Down?"=w496:bool, "Support.Mouse inside icon?"=w497:bool, "Ref.Tools"=w480:refnum<vi>)
          n128 = Equal?(x=lveventtype."Key Repeat", y=w493) -> (x = y?=w491:bool)
          n129 = Equal?(x=w493, y=lveventtype."Key Repeat?" ("x")) -> (x = y?=w492:bool)
          n130 = Or(x=w491, y=w492) -> (x .or. y?=w490:bool)
          n131 = case shown="\"Tool\"" w488 {
            tunnel: w480 -> [_ w570 _]
            tunnel: w500 -> [w507 w572 w667]
            tunnel: w481 -> [w505 w569 w665]
            tunnel: [w503 w568 w664] -> w498
            tunnel: [w506 w571 w666] -> w499
            tunnel: w497 -> [_ w567 _]
            tunnel: w496 -> [_ w566 _]
            tunnel: w482 -> [_ w565 w662]
            tunnel: w489 -> [_ w564 w660]
            tunnel: w487 -> [w504 w562 w663]
            tunnel: [w501 w561 w661] -> w485
            tunnel: w484 -> [w502 _ _]
            tunnel: w483 -> [_ w560 _]
            frame "Default", Default {
              n132 = case shown="\"V\", \"v\"" w504 {
                tunnel: w505 -> [w513 w543 w551 w557]
                tunnel: w507 -> [w516 w544 w553 w559]
                tunnel: [w512 w543 w545 w554] -> w503
                tunnel: [w514 w544 w552 w558] -> w506
                tunnel: [w508 _ w549 w555] -> w501
                tunnel: w502 -> [w509 _ _ _]
                frame "V", "v" {
                  # "Paste"
                  n133 = call "IE Read from Clipboard.vi"("error in"=w516, "Data in"=w513) -> ("error out"=w515:errorcluster, "Data out"=w511:T2, "Empty Clipboard string?"=w510:bool, "Key Focus"=w508:bool)  [unwired: 6 in]
                  n134 = case shown="True" w510 {
                    tunnel: [w518 w524] -> w512
                    tunnel: w511 -> [w517 w525]
                    tunnel: w515 -> [w521 w530]
                    tunnel: [w521 w528] -> w514
                    tunnel: w509 -> [_ w522]
                    frame False {
                      w520 = u32 111  # Invalid tool value
                      w519 = FALSE ("Support.CTRL Pressed")
                      n135 = Bundle By Name(cluster=w517, "Support.Shift pressed?"=w519, "Support.CTRL Pressed"=w519, "Support.Tool (old value)"=w520) -> (w518:T2)
                    }
                    frame True {
                      n136 = call "Empty Picture"() -> ("empty picture"=w527:picture)
                      n137 = call "Import_Clipboard.vi"("error in (no error)"=w530, "Picture in"=w527) -> ("error out"=w529:errorcluster, "Valid?"=w526:bool, "Picture"=w523:picture)  [unwired: 1 in, 6 out]
                      n138 = case shown="True" w526 {
                        tunnel: w525 -> [w531 w537]
                        tunnel: [w531 w533] -> w524
                        tunnel: w529 -> [w532 w542]
                        tunnel: w523 -> [_ w538]
                        tunnel: [w532 w539] -> w528
                        tunnel: w522 -> [_ w535]
                        frame False {
                        }
                        frame True {
                          n139 = call "Create new layer_LayerName_Picture.vi"("error in"=w542, "Layer name"=w535, "Picture"=w538, "Data in"=w537) -> ("error out"=w541:errorcluster, "Data out"=w536:T2)  [unwired: 6 in]
                          n140 = call "ViewLayer.vi"("error in (no error)"=w541, "Data in"=w536) -> ("error out"=w540:errorcluster, "Data out"=w534:T2)  [unwired: 2 in, 6 out]
                          n141 = call "Set Undo Flag.vi"("error in"=w540, "Data in"=w534) -> ("error out"=w539:errorcluster, "Data out"=w533:T2)  [unwired: 8 in]
                        }
                      }
                    }
                  }
                }
                frame Default {
                }
                frame "C", "c" {
                  w548 = u32 111  # Invalid tool value
                  w547 = FALSE ("Support.CTRL Pressed")
                  # "Copy"
                  n142 = call "IE Write to Clipboard.vi"("Is Cut?"=FALSE, "error in"=w553, "Data in"=w551) -> ("error out"=w552:errorcluster, "Key Focus"=w549:bool, "Data out"=w546:T2)  [unwired: 6 in]
                  n143 = Bundle By Name(cluster=w546, "Support.Shift pressed?"=w547, "Support.CTRL Pressed"=w547, "Support.Tool (old value)"=w548) -> (w545:T2)
                }
                frame "X", "x" {
                  # "Cut"
                  n144 = call "IE Write to Clipboard.vi"("Is Cut?"=TRUE, "error in"=w559, "Data in"=w557) -> ("error out"=w558:errorcluster, "Key Focus"=w555:bool, "Data out"=w554:T2)  [unwired: 6 in]
                }
              }
            }
            frame "Tool" {
              n145 = Compound Arithmetic op=AND(invert w566, w567) -> (w563:bool)
              n146 = case shown="Default" w562 {
                tunnel: w570 -> [w582 _ _ _]
                tunnel: w572 -> [w585 w642 w653 w659]
                tunnel: w569 -> [w580 w638 w651 w657]
                tunnel: [w579 w637 w648 w654] -> w568
                tunnel: [w583 w641 w652 w658] -> w571
                tunnel: w563 -> [w577 _ _ _]
                tunnel: w565 -> [w576 _ _ _]
                tunnel: w564 -> [w575 _ _ _]
                tunnel: [_ w636 w649 w655] -> w561
                tunnel: w560 -> [w574 _ _ _]
                frame Default {
                  n147 = call "IsAntsRectValid.vi"("AntsRect"=w574) -> ("Valid?"=w573:bool)  [unwired: 10 out]
                  n148 = property class="RadioBtnsControl (strict)"(reference=w582, error in=w585) -> (reference out=w578:refnum<vi>, error out=w584:errorcluster, "Value"=w581:T12)
                  n149 = case shown="\"Select\"" w581 {
                    selector: w581 -> [w590 w611 _]
                    tunnel: w584 -> [w594 w617 w635]
                    tunnel: w580 -> [w592 w614 w634]
                    tunnel: [w591 w613 w633] -> w579
                    tunnel: w577 -> [w589 _ _]
                    tunnel: w578 -> [w588 w612 _]
                    tunnel: [w593 w616 w635] -> w583
                    tunnel: w576 -> [w587 w610 w632]
                    tunnel: w575 -> [w586 w609 w631]
                    tunnel: w573 -> [_ w615 _]
                    frame "Pencil", Default {
                      n150 = case shown="True" w589 {
                        tunnel: w592 -> [w598 w603]
                        tunnel: [w597 w606] -> w591
                        tunnel: w590 -> [_ w600]
                        tunnel: w594 -> [w599 w607]
                        tunnel: w588 -> [_ w605]
                        tunnel: [w599 w608] -> w593
                        tunnel: w587 -> [_ w602]
                        tunnel: w586 -> [_ w601]
                        frame False {
                          w596 = u32 111  # Invalid tool value
                          w595 = FALSE ("Support.CTRL Pressed")
                          n151 = Bundle By Name(cluster=w598, "Support.Shift pressed?"=w595, "Support.CTRL Pressed"=w595, "Support.Tool (old value)"=w596) -> (w597:T2)
                        }
                        frame True {
                          n152 = Bundle By Name(cluster=w603, "Support.Shift pressed?"=w602, "Support.CTRL Pressed"=w601, "Support.Tool (old value)"=w600) -> (w606:T2)
                          n153 = property class="RadioBtnsControl (strict)"(reference=w605, error in=w607, "Val(Sgnl)"=T12."Dropper" ("Value (Signaling)")) -> (error out=w608:errorcluster)  [unwired: 1 out]
                        }
                      }
                    }
                    frame "Select" {
                      n154 = case shown="False" w615 {
                        tunnel: w614 -> [w621 w629]
                        tunnel: [w620 w628] -> w613
                        tunnel: w617 -> [w626 w630]
                        tunnel: [w625 w630] -> w616
                        tunnel: w612 -> [w622 _]
                        tunnel: w611 -> [w624 _]
                        tunnel: w610 -> [w619 _]
                        tunnel: w609 -> [w618 _]
                        frame False {
                          n155 = Bundle By Name(cluster=w621, "Support.Shift pressed?"=w619, "Support.CTRL Pressed"=w618, "Support.Tool (old value)"=w624) -> (w620:T2)
                          n156 = property class="RadioBtnsControl (strict)"(reference=w622, error in=w626, "Val(Sgnl)"=T12."Dropper" ("Value (Signaling)")) -> (error out=w625:errorcluster)  [unwired: 1 out]
                        }
                        frame True {
                          w627 = u32 111  # Invalid tool value
                          n157 = Bundle By Name(cluster=w629, "Support.Tool (old value)"=w627) -> (w628:T2)
                        }
                      }
                    }
                    frame "Dropper" {
                      n158 = Bundle By Name(cluster=w634, "Support.Shift pressed?"=w632, "Support.CTRL Pressed"=w631) -> (w633:T2)
                    }
                  }
                }
                frame "V", "v" {
                  # "Paste"
                  n159 = call "IE Read from Clipboard.vi"("error in"=w642, "Data in"=w638) -> ("error out"=w641:errorcluster, "Data out"=w640:T2, "Empty Clipboard string?"=w639:bool, "Key Focus"=w636:bool)  [unwired: 6 in]
                  n160 = case shown="False" w639 {
                    tunnel: [w644 w647] -> w637
                    tunnel: w640 -> [w643 w647]
                    frame False {
                      w646 = u32 111  # Invalid tool value
                      w645 = FALSE ("Support.CTRL Pressed")
                      n161 = Bundle By Name(cluster=w643, "Support.Shift pressed?"=w645, "Support.CTRL Pressed"=w645, "Support.Tool (old value)"=w646) -> (w644:T2)
                    }
                    frame True {
                    }
                  }
                }
                frame "C", "c" {
                  # "Copy"
                  n162 = call "IE Write to Clipboard.vi"("Is Cut?"=FALSE, "error in"=w653, "Data in"=w651) -> ("error out"=w652:errorcluster, "Key Focus"=w649:bool, "Data out"=w648:T2)  [unwired: 6 in]
                }
                frame "X", "x" {
                  # "Cut"
                  n163 = call "IE Write to Clipboard.vi"("Is Cut?"=TRUE, "error in"=w659, "Data in"=w657) -> ("error out"=w658:errorcluster, "Key Focus"=w655:bool, "Data out"=w654:T2)  [unwired: 6 in]
                }
              }
            }
            frame "Move Selection" {
              n164 = case shown="\"Z\", \"z\"" w663 {
                tunnel: w667 -> [w669 w675 w686]
                tunnel: w665 -> [w668 w673 w684]
                tunnel: [w668 w672 w683] -> w664
                tunnel: w662 -> [_ w671 _]
                tunnel: [_ TRUE _] -> w661
                tunnel: [w669 w674 w685] -> w666
                tunnel: w660 -> [_ _ _]
                frame Default {
                }
                frame "Z", "z" {
                  # "Undo"
                  n165 = case shown="False" w671 {
                    tunnel: w675 -> [w680 w682]
                    tunnel: w673 -> [w678 w681]
                    tunnel: [w677 w681] -> w672
                    tunnel: [w679 w682] -> w674
                    frame False {
                      w676 = FALSE  # Reset cursor
                      n166 = call "Escape.vi"("Reset cursor (T)"=w676, "error in"=w680, "Data in"=w678) -> ("error out"=w679:errorcluster, "Data out"=w677:T2)  [unwired: 7 out]
                    }
                    frame True {
                    }
                  }
                }
                frame "V", "v" {
                  # "Paste"
                  n167 = call "Finalize Movement.vi"("error in (no error)"=w686, "Data in"=w684) -> ("error out"=w685:errorcluster, "Data out"=w683:T2)  [unwired: 2 in, 6 out]
                }
              }
            }
          }
          n168 = Or(x=w485, y=w490) -> (x .or. y?=w486:bool)
        }
      }
    }
    frame Error {
    }
  }
  "error out" <- w9
  "Discard?" <- w5
  "Data out" <- w3
